vi "Create Element.vi"(8 "error in":errorcluster, 9 "Type Definitions Folder":path, 10 "Parameter":T1, 11 "IElement Manager in":refnum<class "IElement Manager.lvclass">) -> (0 "error out":errorcluster, 2 "IElement":refnum<class "IElement.lvclass">, 3 "IElement Manager out":refnum<class "IElement Manager.lvclass">)   [LabVIEW 2026, in "IElement Manager.lvclass"]
doc: "Create element from function parameter cluster."
uses:
  IElement Manager.lvclass
  Type Definitions/Parameter--cluster.ctl
  IElement/IElement.lvclass
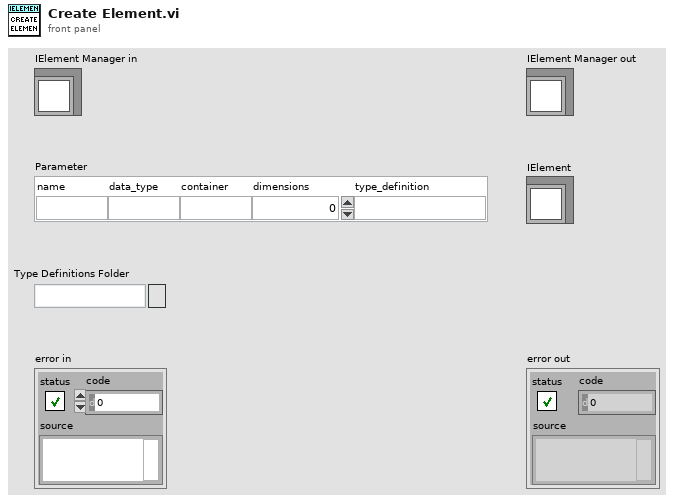
[diagram p1: front panel]
types:
  T1 = typedef "Parameter--cluster.ctl" = cluster{"name":string, "data_type":string, "container":string, "dimensions":i32, "type_definition":string}
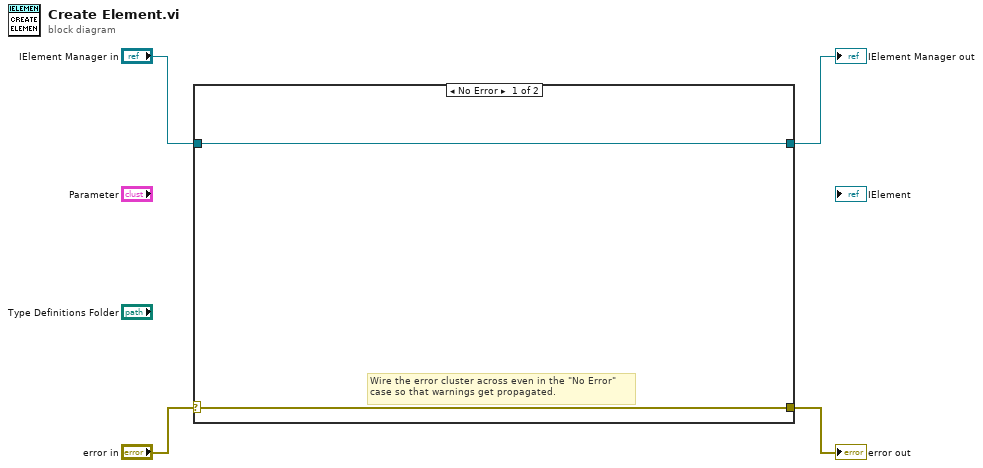
[diagram p0: block diagram]
diagram:
  n1 = case shown="No Error" "error in" {
    selector: "error in" -> [w6 w8]
    tunnel: [w6 w8] -> w3
    tunnel: [w5 w7] -> w1
    tunnel: "IElement Manager in" -> [w5 w7]
    frame No Error {
      # "Wire the error cluster across even in the \"No Error\"\ncase so that warnings get propagated."
    }
    frame Error {
    }
  }
  "error out" <- w3
  "IElement Manager out" <- w1
